vi "MecaDrivePoseEst_New.vi"(4 "WheelPositions":T1 {"RearRight" format="%19.3f"; "RearLeft" format="%19.3f"; "FrontRight" format="%19.3f"; "FrontLeft" format="%19.3f"}, 5 "gyroAngle":T6={"VALUE"=0.0, "COS"=1.0, "SIN"=0.0} {"SIN" format="%13.4f"; "COS" format="%13.4f"; "VALUE" format="%13.4f"}, 6 "MecanumKinematics":T2={"FrontLeft"={"X"=0.0, "Y"=0.0}, "FrontRight"={"X"=0.0, "Y"=0.0}, "RearLeft"={"X"=0.0, "Y"=0.0}, "RearRight"={"X"=0.0, "Y"=0.0}, "InverseKinematics"=[[0.0, 1.0, -1.0, 0.0], [0.0, 1.0, 1.0, 0.0], [0.0, 1.0, 1.0, 0.0], [0.0, 1.0, -1.0, 0.0]], "ForwardKinematics"=[[0.0, 1.0, -1.0, 0.0], [0.0, 1.0, 1.0, 0.0], [0.0, 1.0, 1.0, 0.0], [0.0, 1.0, -1.0, 0.0]], "PrevCoR"={"X"=0.0, "Y"=0.0}} {"PrevCoR"."Y" format="%14.3f"; "PrevCoR"."X" format="%14.3f"; "RearRight"."Y" format="%14.3f"; "RearRight"."X" format="%14.3f"; "RearLeft"."Y" format="%14.3f"; "RearLeft"."X" format="%14.3f"; "FrontRight"."Y" format="%14.3f"; "FrontRight"."X" format="%14.3f"; "FrontLeft"."Y" format="%14.3f"; "FrontLeft"."X" format="%14.3f"}, 7 "InitialPose":T5={"TRANSLATION"={"X"=0.0, "Y"=0.0}, "ROTATION"={"VALUE"=0.0, "COS"=1.0, "SIN"=0.0}} {"ROTATION"."SIN" format="%13.4f"; "ROTATION"."COS" format="%13.4f"; "ROTATION"."VALUE" format="%13.4f"; "TRANSLATION"."Y" format="%14.3f"; "TRANSLATION"."X" format="%14.3f"}, 8 "dt_Seconds":dbl=0.02, 9 "VisionMeasurementStdDevs":T4=[[0.0], [0.0], [0.0]], 10 "LocalMeasurementStdDevs":T4=[[0.0], [0.0], [0.0], [0.0], [0.0]], 11 "StateStdDevs":T4=[[0.0], [0.0], [0.0], [0.0], [0.0], [0.0], [0.0]]) -> (0 "Error":errorcluster, 3 "MecaDrivePoseEstimate":T7={"M_VisionContR"=[], "m_nominal_dT"=0.0, "m_PrevTime_Sec"=0.0, "m_GyroOffset"={"VALUE"=0.0, "COS"=1.0, "SIN"=0.0}, "m_PrevAngle"={"VALUE"=0.0, "COS"=1.0, "SIN"=0.0}, "m_Observer"={"m_P"=[], "m_xHat"=[], "States"=0, "Outputs"=0, "m_ContR"=[], "m_ContQ"=[], "m_SigmasF"=[], "m_dT_Sec"=0.0, "MERWE_SCALED_SIGMA_PTS"={"m_Wm"=[], "States"=0, "Alpha"=0.0, "m_Wc"=[], "Kappa"=0}, "meanFuncX"=refnum, "meanFuncY"=refnum, "residualFuncX"=refnum, "residualFuncY"=refnum, "addFuncX"=refnum, "addFuncXExtra"=variant, "residualFuncYExtra"=variant, "residualFuncXExtra"=variant, "MeanFuncYExtra"=variant, "MeanFuncXExtra"=variant, "Inputs"=0}, "m_kinematics"={"FrontLeft"={"X"=0.0, "Y"=0.0}, "FrontRight"={"X"=0.0, "Y"=0.0}, "RearLeft"={"X"=0.0, "Y"=0.0}, "RearRight"={"X"=0.0, "Y"=0.0}, "InverseKinematics"=[[0.0, 1.0, -1.0, 0.0], [0.0, 1.0, 1.0, 0.0], [0.0, 1.0, 1.0, 0.0], [0.0, 1.0, -1.0, 0.0]], "ForwardKinematics"=[[0.0, 1.0, -1.0, 0.0], [0.0, 1.0, 1.0, 0.0], [0.0, 1.0, 1.0, 0.0], [0.0, 1.0, -1.0, 0.0]], "PrevCoR"={"X"=0.0, "Y"=0.0}}, "Pose_Buffer"={"TimeStamps"=[], "Pose"=[], "Min_TimeStamp"=0.0, "Max_TimeStamp"=0.0, "ItemCount"=0, "MaxBufferTime"=0.0}} {"Pose_Buffer"."Pose"."ROTATION"."SIN" format="%13.4f"; "Pose_Buffer"."Pose"."ROTATION"."COS" format="%13.4f"; "Pose_Buffer"."Pose"."ROTATION"."VALUE" format="%13.4f"; "Pose_Buffer"."Pose"."TRANSLATION"."Y" format="%14.3f"; "Pose_Buffer"."Pose"."TRANSLATION"."X" format="%14.3f"; "m_kinematics"."PrevCoR"."Y" format="%14.3f"; "m_kinematics"."PrevCoR"."X" format="%14.3f"; "m_kinematics"."RearRight"."Y" format="%14.3f"; "m_kinematics"."RearRight"."X" format="%14.3f"; "m_kinematics"."RearLeft"."Y" format="%14.3f"; "m_kinematics"."RearLeft"."X" format="%14.3f"; "m_kinematics"."FrontRight"."Y" format="%14.3f"; "m_kinematics"."FrontRight"."X" format="%14.3f"; "m_kinematics"."FrontLeft"."Y" format="%14.3f"; "m_kinematics"."FrontLeft"."X" format="%14.3f"; "m_PrevAngle"."SIN" format="%13.4f"; "m_PrevAngle"."COS" format="%13.4f"; "m_PrevAngle"."VALUE" format="%13.4f"; "m_GyroOffset"."SIN" format="%13.4f"; "m_GyroOffset"."COS" format="%13.4f"; "m_GyroOffset"."VALUE" format="%13.4f"})   [LabVIEW 2019, in "Trajectory_Library.lvlib"]
doc: "Constructs a MecaDrivePoseEstimator.\n\nThis data cluster and its associated function blocks wrap an UnscentedKalmanFilter Unscented Kalman Filter to fuse latency-compensated vision measurements with mecanum drive encoder velocity measurements. It will correct for noisy measurements and encoder drift. It is intended to be an easy but more accurate drop-in for MecanumDriveOdometry.\n \nMecanumDrivePoseEstimator_update should be called every robot loop. If your loops are faster or slower than the default of 20 ms, then you should change the nominal delta time using the secondary constructor: MecanumDrivePoseEstimator_MecanumDrivePoseEstimator(Rotation2d, Pose2d MecanumDriveWheelPositions, MecanumDriveKinematics, Matrix, Matrix, Matrix, double).\n \nMecanumDrivePoseEstimator_addVisionMeasurement can be called as infrequently as you want; if you never call it, then this data cluster will behave mostly like regular encoder odometry.\n \nThe state-space system used internally has the following states (x), inputs (u), and outputs (y):\n \n x = [x, y, theta, s_fl, s_fr, s_rl, s_rr]T \n\n in the field coordinate system containing x position, y position, and heading, followed by\n the distance driven by the front left, front right, rear left, and rear right wheels.\n \n u = [v_x, v_y, omega, v_fl, v_fr, v_rl, v_rr]T \n\n containing x velocity, y velocity, and angular rate in the field coordinate system, \n followed by the velocity of the front left, front right, rear left, and rear right wheels.\n \n y = [x, y, theta]T \n\n from vision containing x position, y position, and heading; or \n\n y = [theta, s_fl, s_fr, s_rl, s_rr]T\n\n containing gyro heading, followed by the distance driven by the front left, front \n right, rear left, and rear right wheels.\n \nInputs: \n - gyroAngle -- The current gyro angle.\n - initialPoseMeters -- The starting pose estimate.\n - wheelPositions -- The distances driven by each wheel.\n - kinematics -- A correctly-configured kinematics object for your drivetrain.\n - stateStdDevs -- Standard deviations of model states. Increase these numbers\n to trust your model's state estimates less. This matrix is in the\n form [x, y, theta, s_fl, s_fr, s_rl, s_rr]T, with units in meters \n and radians, followed by meters.\n - localMeasurementStdDevs -- Standard deviation of the gyro measurement. \n Increase this number to trust sensor readings from the gyro less. \n This matrix is in the form [theta, s_fl, s_fr, s_rl, s_rr], with \n units in radians, followed by meters.\n - visionMeasurementStdDevs -- Standard deviations of the vision measurements. \n Increase these numbers to trust global measurements from vision \n less. This matrix is in the form [x, y, theta]T, with units in \n meters and radians.\n - nominalDtSeconds -- The time in seconds between each robot loop.\n\nOutputs:\n - outMecaPoseEst -- Updated data cluster \n - Error -- If TRUE, an error occured."
uses:
  Trajectory_Library.lvlib
  <vilib>/Analysis/Matrix/Datatypes/RealMatrix.ctl
  <vilib>/Analysis/Matrix/NI_Matrix.lvlib
  TypeDef/MERWE_SCALED_SIGMA_PTS.ctl
  TypeDef/UNSCENTED_KALMAN_FILTER.ctl
  TypeDef/CALLBACK_FUNC_TYPE.ctl
  TypeDef/ROTATION2D.ctl
  TypeDef/TRANSLATION2D.ctl
  TypeDef/POSE2D.ctl
  TypeDef/TIME_INTERPOLATABLE_POSE2D.ctl
  TypeDef/MECA_DRIVE_KINEMATICS.ctl
  TypeDef/MECA_DRIVE_POSE_EST.ctl
  TypeDef/MECA_WHEEL_POSITIONS.ctl
panel:
  # "<7,1>"
  # "<5, 1>"
  # "<3, 1>"
  # "<3, 3>"
  # "State Estimate <Statess,1>"
  # "<States, States>"
  # "<States, ?>"
  # "<Statess,  States>"
  # "<Outputs, Outputs>"
  # "<?, 1>"
  # "<?, 1>"
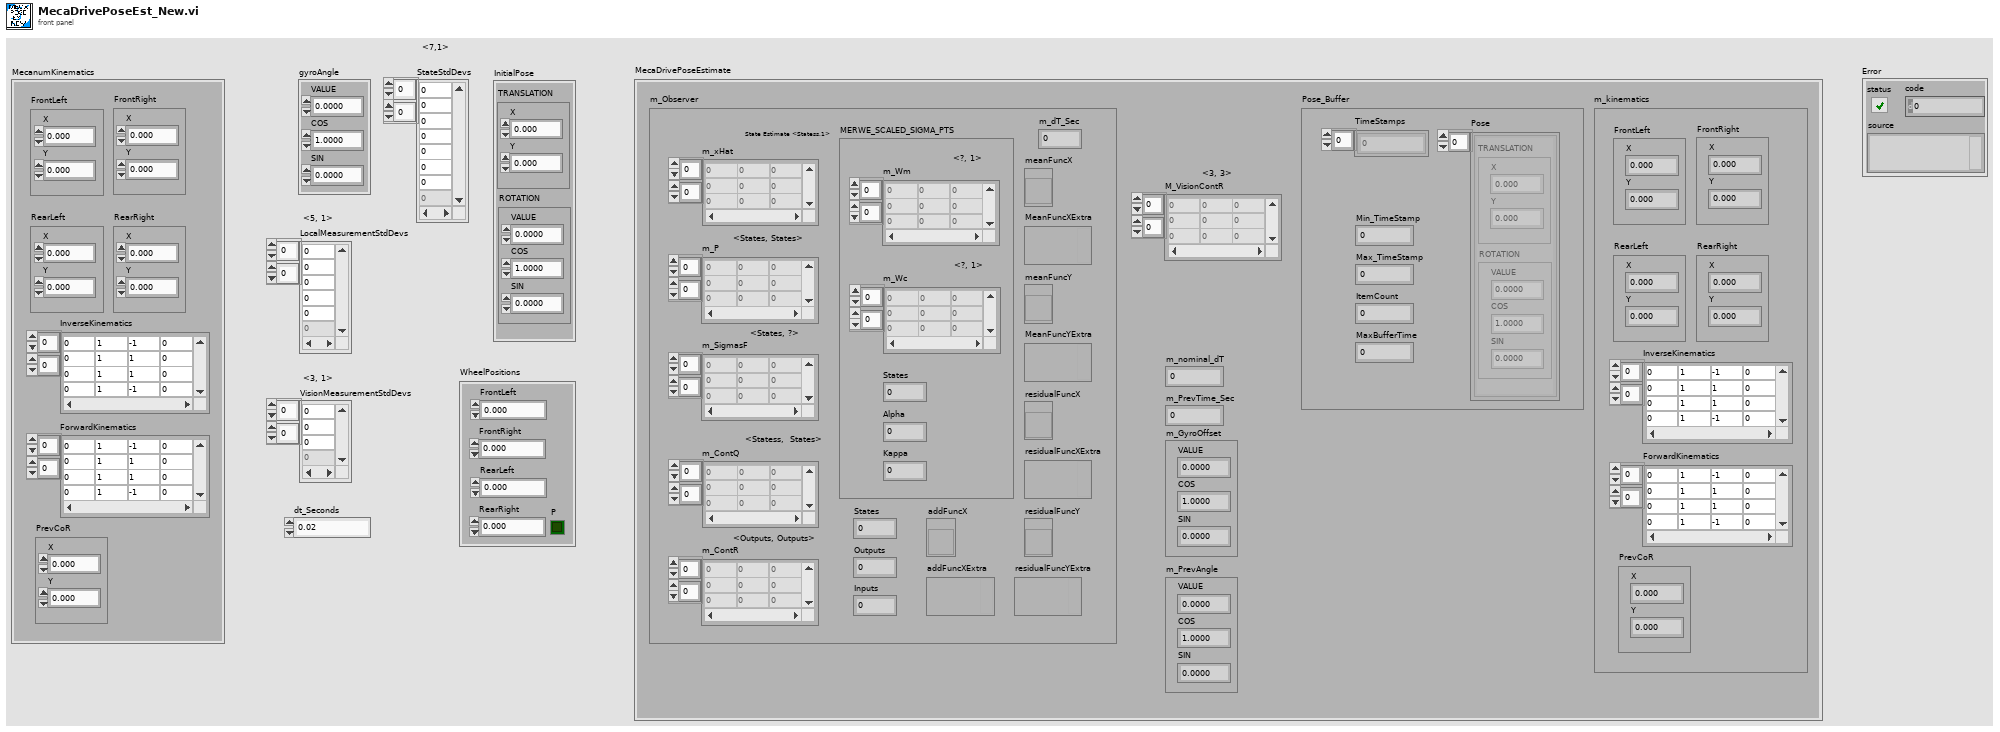
[diagram p1: front panel]
types:
  T1 = typedef "Trajectory_Library.lvlib/MECA_WHEEL_POSITIONS.ctl" = cluster{"FrontLeft":dbl, "FrontRight":dbl, "RearLeft":dbl, "RearRight":dbl, "P":bool}
  T2 = typedef "Trajectory_Library.lvlib/MECA_DRIVE_KINEMATICS.ctl" = cluster{"FrontLeft":T3, "FrontRight":T3, "RearLeft":T3, "RearRight":T3, "InverseKinematics":T4, "ForwardKinematics":T4, "PrevCoR":T3}
  T3 = typedef "Trajectory_Library.lvlib/TRANSLATION2D.ctl" = cluster{"X":dbl, "Y":dbl}
  T4 = typedef "NI_Matrix.lvlib/RealMatrix.ctl" = dbl[][]
  T5 = typedef "Trajectory_Library.lvlib/POSE2D.ctl" = cluster{"TRANSLATION":T3, "ROTATION":T6}
  T6 = typedef "Trajectory_Library.lvlib/ROTATION2D.ctl" = cluster{"VALUE":dbl, "COS":dbl, "SIN":dbl}
  T7 = typedef "Trajectory_Library.lvlib/MECA_DRIVE_POSE_EST.ctl" = cluster{"M_VisionContR":T4, "m_nominal_dT":dbl, "m_PrevTime_Sec":dbl, "m_GyroOffset":T6, "m_PrevAngle":T6, "m_Observer":T8, "m_kinematics":T2, "Pose_Buffer":T11}
  T8 = typedef "Trajectory_Library.lvlib/UNSCENTED_KALMAN_FILTER.ctl" = cluster{"m_P":T4, "m_xHat":T4, "States":i32, "Outputs":i32, "m_ContR":T4, "m_ContQ":T4, "m_SigmasF":T4, "m_dT_Sec":dbl, "MERWE_SCALED_SIGMA_PTS":T9, "meanFuncX":T10, "meanFuncY":T10, "residualFuncX":T10, "residualFuncY":T10, "addFuncX":T10, "addFuncXExtra":variant, "residualFuncYExtra":variant, "residualFuncXExtra":variant, "MeanFuncYExtra":variant, "MeanFuncXExtra":variant, "Inputs":i32}
  T9 = typedef "Trajectory_Library.lvlib/MERWE_SCALED_SIGMA_PTS.ctl" = cluster{"m_Wm":T4, "States":i32, "Alpha":dbl, "m_Wc":T4, "Kappa":i32}
  T10 = typedef "Trajectory_Library.lvlib/CALLBACK_FUNC_TYPE.ctl" = refnum<vi>
  T11 = typedef "Trajectory_Library.lvlib/TIME_INTERPOLATABLE_POSE2D.ctl" = cluster{"TimeStamps":dbl[], "Pose":T5[], "Min_TimeStamp":dbl, "Max_TimeStamp":dbl, "ItemCount":i32, "MaxBufferTime":dbl}
  T12 = typedef "Trajectory_Library.lvlib/UNSCENTED_KALMAN_NEW_FUNC_GROUP.ctl" = cluster{"meanFuncX":T10, "meanFuncY":T10, "residualFuncX":T10, "residualFuncY":T10, "addFuncX":T10, "MeanFuncXExtra":variant, "MeanFuncYExtra":variant, "residualFuncXExtra":variant, "residualFuncYExtra":variant, "addFuncXExtra":variant}
  T13 = typedef "WPILib_Math.lvlib/TIME_INTERPOLATABLE_POSE2D.ctl" = cluster{"TimeStamps":dbl[], "Pose":T14[], "Min_TimeStamp":dbl, "Max_TimeStamp":dbl, "ItemCount":i32, "MaxBufferTime":dbl}
  T14 = typedef "WPILib_Math.lvlib/POSE2D.ctl" = cluster{"TRANSLATION":T15, "ROTATION":T16}
  T15 = typedef "WPILib_Math.lvlib/TRANSLATION2D.ctl" = cluster{"X":dbl, "Y":dbl}
  T16 = typedef "WPILib_Math.lvlib/ROTATION2D.ctl" = cluster{"VALUE":dbl, "COS":dbl, "SIN":dbl}
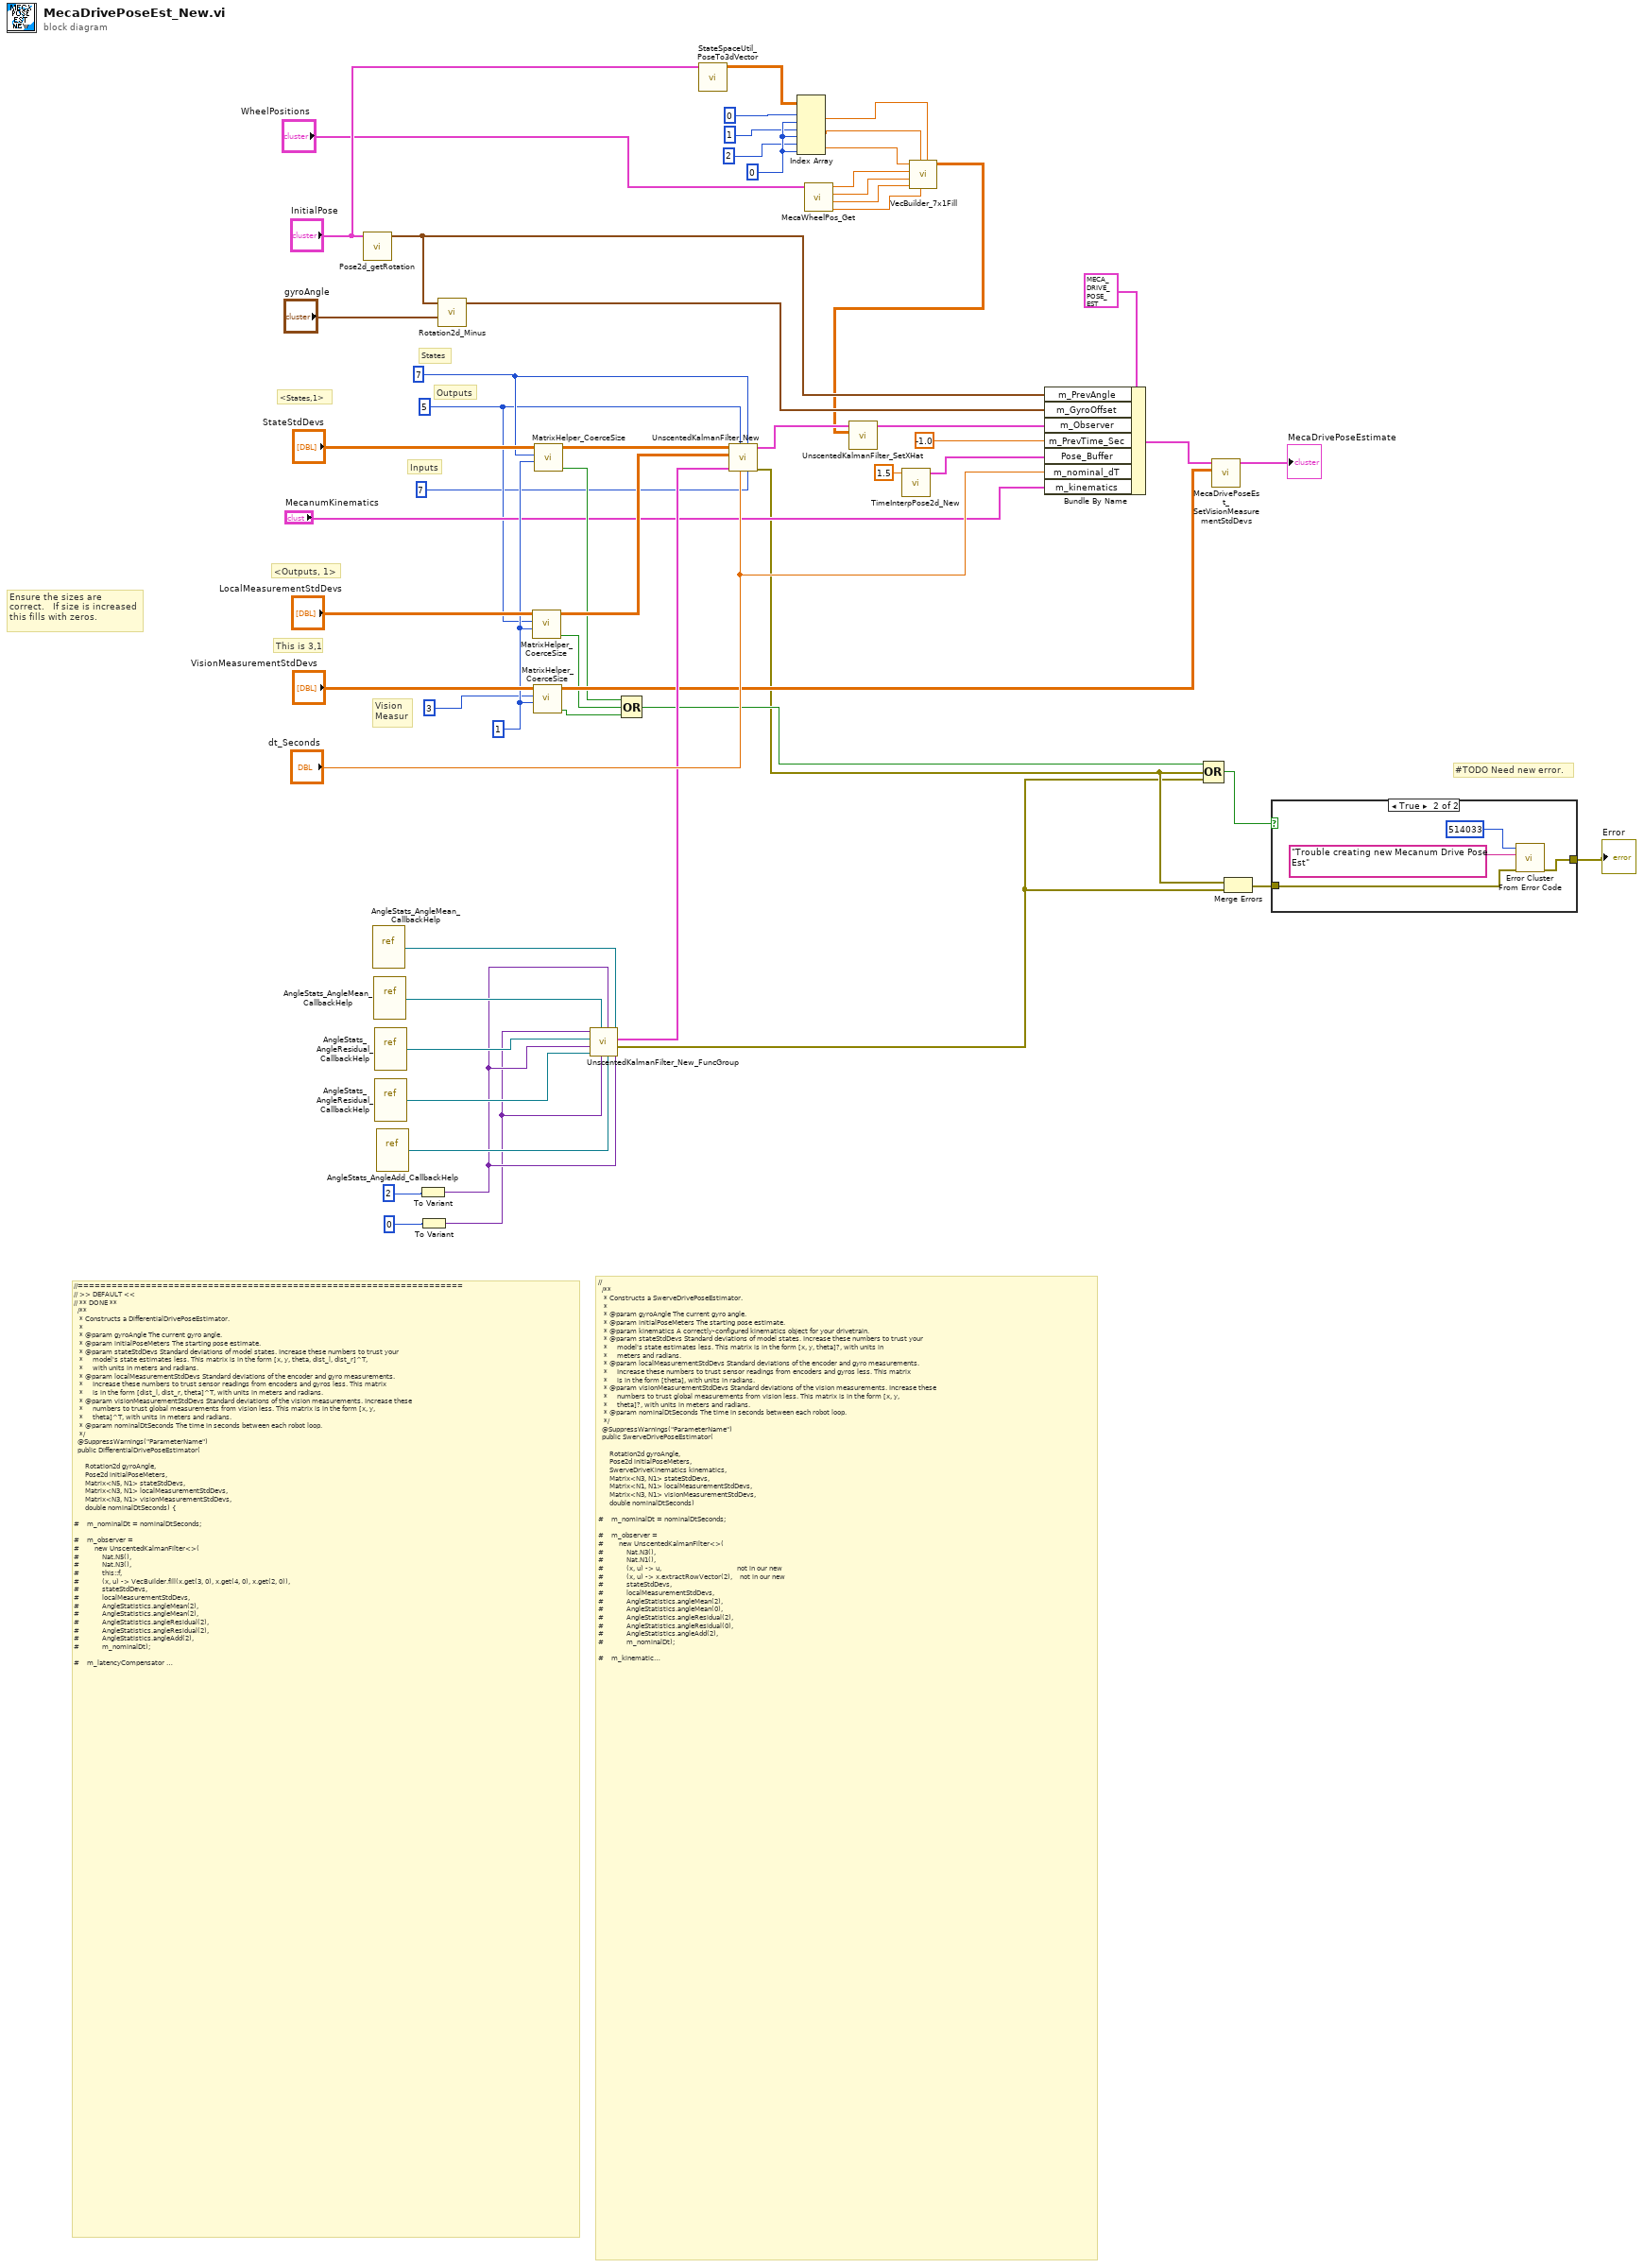
[diagram p0: block diagram]
diagram:
  w12 = 0 ("index (col)")
  w34 = 1 ("y")
  w25 = 5 ("Outputs")
  w33 = 7 ("States")
  # "Vision\nMeasur"
  # "#TODO Need new error."
  # "This is 3,1"
  # "//====================================================================\n// >> DEFAULT <<\n// ** DONE **\n  /**\n   * Constructs a DifferentialDrivePoseEstimator.\n   *\n   * @param gyroAngle The current gyro angle.\n   * @param initialPoseMeters The starting pose estimate.\n   * @param stateStdDevs Standard deviations of model states. Increase these numbers to trust your\n   *     model's state estimates less. This matrix is in the form [x, y, theta, dist_l, dist_r]^T,\n   *     with units in meters and radians.\n   * @param localMeasurementStdDevs Standard deviations of the encoder and gyro measurements.\n   *     Increase these numbers to trust sensor readings from encoders and gyros less. This matrix\n   *     is in the form [dist_l, dist_r, theta]^T, with units in meters and radians.\n   * @param visionMeasurementStdDevs Standard deviations of the vision measurements. Increase these\n   *     numbers to trust global measurements from vision less. This matrix is in the form [x, y,\n   *     theta]^T, with units in meters and radians.\n   * @param nominalDtSeconds The time in seconds between each robot loop.\n   */\n  @SuppressWarnings(\"ParameterName\")\n  public DifferentialDrivePoseEstimator(\n\n      Rotation2d gyroAngle,\n      Pose2d initialPoseMeters,\n      Matrix<N5, N1> stateStdDevs,\n      Matrix<N3, N1> localMeasurementStdDevs,\n      Matrix<N3, N1> visionMeasurementStdDevs,\n      double nominalDtSeconds) {\n\n#    m_nominalDt = nominalDtSeconds;\n\n#    m_observer =\n#        new UnscentedKalmanFilter<>(\n#            Nat.N5(),\n#            Nat.N3(),\n#            this::f,\n#            (x, u) -> VecBuilder.fill(x.get(3, 0), x.get(4, 0), x.get(2, 0)),\n#            stateStdDevs,\n#            localMeasurementStdDevs,\n#            AngleStatistics.angleMean(2),\n#            AngleStatistics.angleMean(2),\n#            AngleStatistics.angleResidual(2),\n#            AngleStatistics.angleResidual(2),\n#            AngleStatistics.angleAdd(2),\n#            m_nominalDt);\n\n#    m_latencyCompensator = new KalmanFilterLatencyCompensator<>();\n\n#    // Initialize vision R\n#    setVisionMeasurementStdDevs(visionMeasurementStdDevs);\n\n//JAS not part of the data structure....\n    m_visionCorrect =\n        (u, y) ->\n            m_observer.correct(\n                Nat.N3(),\n                u,\n                y,\n                (x, u1) -> new Matrix<>(x.getStorage().extractMatrix(0, 3, 0, 1)),\n                m_visionDiscreteR,\n                AngleStatistics.angleMean(2),\n                AngleStatistics.angleResidual(2),\n                AngleStatistics.angleResidual(2),\n                AngleStatistics.angleAdd(2));\n\n#    m_gyroOffset = initialPoseMeters.getRotation().minus(gyroAngle);\n#    m_previousAngle = initialPoseMeters.getRotation();\n#    m_observer.setXhat(fillStateVector(initialPoseMeters, 0.0, 0.0));\n  }"
  # "// \n  /**\n   * Constructs a SwerveDrivePoseEstimator.\n   *\n   * @param gyroAngle The current gyro angle.\n   * @param initialPoseMeters The starting pose estimate.\n   * @param kinematics A correctly-configured kinematics object for your drivetrain.\n   * @param stateStdDevs Standard deviations of model states. Increase these numbers to trust your\n   *     model's state estimates less. This matrix is in the form [x, y, theta]?, with units in\n   *     meters and radians.\n   * @param localMeasurementStdDevs Standard deviations of the encoder and gyro measurements.\n   *     Increase these numbers to trust sensor readings from encoders and gyros less. This matrix\n   *     is in the form [theta], with units in radians.\n   * @param visionMeasurementStdDevs Standard deviations of the vision measurements. Increase these\n   *     numbers to trust global measurements from vision less. This matrix is in the form [x, y,\n   *     theta]?, with units in meters and radians.\n   * @param nominalDtSeconds The time in seconds between each robot loop.\n   */\n  @SuppressWarnings(\"ParameterName\")\n  public SwerveDrivePoseEstimator(\n\n      Rotation2d gyroAngle,\n      Pose2d initialPoseMeters,\n      SwerveDriveKinematics kinematics,\n      Matrix<N3, N1> stateStdDevs,\n      Matrix<N1, N1> localMeasurementStdDevs,\n      Matrix<N3, N1> visionMeasurementStdDevs,\n      double nominalDtSeconds) \n\n#    m_nominalDt = nominalDtSeconds;\n\n#    m_observer =\n#        new UnscentedKalmanFilter<>(\n#            Nat.N3(),\n#            Nat.N1(),\n#            (x, u) -> u,                                        not in our new\n#            (x, u) -> x.extractRowVector(2),    not in our new\n#            stateStdDevs,\n#            localMeasurementStdDevs,\n#            AngleStatistics.angleMean(2),\n#            AngleStatistics.angleMean(0),\n#            AngleStatistics.angleResidual(2),\n#            AngleStatistics.angleResidual(0),\n#            AngleStatistics.angleAdd(2),\n#            m_nominalDt);\n\n#    m_kinematics = kinematics;\n\n#    m_latencyCompensator = new KalmanFilterLatencyCompensator<>();\n\n#    // Initialize vision R\n#    setVisionMeasurementStdDevs(visionMeasurementStdDevs);\n\n//JAS not part of the data structure....\n    m_visionCorrect =\n        (u, y) ->\n            m_observer.correct(\n                Nat.N3(),\n                u,\n                y,\n                (x, u1) -> x,\n                m_visionContR,\n                AngleStatistics.angleMean(2),\n                AngleStatistics.angleResidual(2),\n                AngleStatistics.angleResidual(2),\n                AngleStatistics.angleAdd(2));\n\n#    m_gyroOffset = initialPoseMeters.getRotation().minus(gyroAngle);\n#    m_previousAngle = initialPoseMeters.getRotation();\n#    m_observer.setXhat(  StateSpaceUtil.poseTo3dVector(initialPoseMeters));\n  }"
  # "Inputs"
  # "Outputs"
  # "States"
  # "<Outputs, 1>"
  # "<States,1>"
  # "Ensure the sizes are\ncorrect.   If size is increased \nthis fills with zeros."
  n1 = call "Pose2d_getRotation.vi"("in POSE"="InitialPose") -> ("out ROTATION"=w54:T6)  [unwired: 10 in]
  n2 = vi-ref "AngleStats_AngleMean_CallbackHelp.vi"() -> (w47:refnum<vi>)
  n3 = vi-ref "AngleStats_AngleMean_CallbackHelp.vi"() -> (w46:refnum<vi>)
  n4 = vi-ref "AngleStats_AngleResidual_CallbackHelp.vi"() -> (w45:refnum<vi>)
  n5 = vi-ref "AngleStats_AngleResidual_CallbackHelp.vi"() -> (w44:refnum<vi>)
  n6 = vi-ref "AngleStats_AngleAdd_CallbackHelp.vi"() -> (w42:refnum<vi>)
  n7 = To Variant(anything=2) -> (Variant=w41:variant)
  n8 = To Variant(anything=0) -> (Variant=w27:variant)
  n9 = call "Rotation2d_Minus.vi"("other ROTATION"="gyroAngle", "in ROTATION"=w54) -> ("out ROTATION"=w55:T6)  [unwired: 9 in]
  n10 = call "MatrixHelper_CoerceSize.vi"("Columns"=w34, "Rows"=w25, "input matrix"="LocalMeasurementStdDevs") -> ("Coerced"=w30:bool, "output matrix"=w39:T4)  [unwired: 7 in]
  n11 = call "MatrixHelper_CoerceSize.vi"("Columns"=w34, "Rows"=3 ("Inputs"), "input matrix"="VisionMeasurementStdDevs") -> ("Coerced"=w29:bool, "output matrix"=w35:T4)  [unwired: 7 in]
  n12 = call "MatrixHelper_CoerceSize.vi"("Columns"=w34, "Rows"=w33, "input matrix"="StateStdDevs") -> ("Coerced"=w31:bool, "output matrix"=w37:T4)  [unwired: 7 in]
  n13 = call "UnscentedKalmanFilter_New_FuncGroup.vi"("addFuncXExtra"=w41, "MeanFuncX"=w47, "AddFuncX"=w42, "MeanFuncXExtra"=w41, "residualFuncYExtra"=w27, "MeanFuncY"=w46, "ResidualFuncY"=w44, "residualFuncXExtra"=w41, "ResidualFuncX"=w45, "MeanFuncYExtra"=w27) -> ("Error"=w19:errorcluster, "UNSCENTED_KALMAN_NEW_FUNC_GROUP"=w48:T12)
  n14 = Compound Arithmetic op=OR(w31, w30, w29) -> (w32:bool)
  n15 = call "StateSpaceUtil_PoseTo3dVector.vi"("Pose"="InitialPose") -> ("Pose Vector"=w14:T4)  [unwired: 10 in]
  n16 = call "UnscentedKalmanFilter_New.vi"("Inputs"=7, "States"=w33, "dt_Seconds"="dt_Seconds", "Outputs"=w25, "UNSCENTED_KALMAN_NEW_FUNC_GROUP"=w48, "MeasurementStdDevs"=w39, "StateStdDevs"=w37) -> ("Error"=w20:errorcluster, "UnscentedKalmanFiilter"=w52:T8)  [unwired: 3 in]
  n17 = Index Array(array=w14, index (row) #1=0 ("index (row)"), index (col) #1=w12, index (row) #2=1 ("index (row)"), index (col) #2=w12, index (row) #3=2 ("index (row)"), index (col) #3=w12) -> (element #1=w9:dbl, element #2=w8:dbl, element #3=w7:dbl)
  n18 = call "MecaWheelPos_Get.vi"("MECA_WHEEL_POSITIONS"="WheelPositions") -> ("RearRightPosition"=w3:dbl, "RearLeftPosition"=w4:dbl, "FrontRightPosition"=w5:dbl, "FrontLeftPosition"=w6:dbl)  [unwired: 7 in]
  n19 = call "TimeInterpPose2d_New.vi"("MaxTime"=1.5) -> ("TimeInterpPose"=w16:T13)  [unwired: 10 in]
  n20 = call "VecBuilder_7x1Fill.vi"("R0"=w9, "R6"=w3, "R1"=w8, "R5"=w4, "R4"=w5, "R3"=w6, "R2"=w7) -> ("output matrix"=w1:T4)  [unwired: 4 in]
  n21 = call "UnscentedKalmanFilter_SetXHat.vi"("xHat"=w1, "in UnscentedKalmanFiilter"=w52) -> ("out UnscentedKalmanFiilter"=w53:T8)  [unwired: 8 in, 1 out]
  n22 = Bundle By Name(cluster=T7 {"M_VisionContR"=[], "m_nominal_dT"=0.0, "m_PrevTime_Sec"=0.0, "m_GyroOffset"={"VALUE"=0.0, "COS"=1.0, "SIN"=0.0}, "m_PrevAngle"={"VALUE"=0.0, "COS"=1.0, "SIN"=0.0}, "m_Observer"={"m_P"=[], "m_xHat"=[], "States"=0, "Outputs"=0, "m_ContR"=[], "m_ContQ"=[], "m_SigmasF"=[], "m_dT_Sec"=0.0, "MERWE_SCALED_SIGMA_PTS"={"m_Wm"=[], "States"=0, "Alpha"=0.0, "m_Wc"=[], "Kappa"=0}, "meanFuncX"=refnum, "meanFuncY"=refnum, "residualFuncX"=refnum, "residualFuncY"=refnum, "addFuncX"=refnum, "addFuncXExtra"=variant, "residualFuncYExtra"=variant, "residualFuncXExtra"=variant, "MeanFuncYExtra"=variant, "MeanFuncXExtra"=variant, "Inputs"=0}, "m_kinematics"={"FrontLeft"={"X"=0.0, "Y"=0.0}, "FrontRight"={"X"=0.0, "Y"=0.0}, "RearLeft"={"X"=0.0, "Y"=0.0}, "RearRight"={"X"=0.0, "Y"=0.0}, "InverseKinematics"=[[0.0, 1.0, -1.0, 0.0], [0.0, 1.0, 1.0, 0.0], [0.0, 1.0, 1.0, 0.0], [0.0, 1.0, -1.0, 0.0]], "ForwardKinematics"=[[0.0, 1.0, -1.0, 0.0], [0.0, 1.0, 1.0, 0.0], [0.0, 1.0, 1.0, 0.0], [0.0, 1.0, -1.0, 0.0]], "PrevCoR"={"X"=0.0, "Y"=0.0}}, "Pose_Buffer"={"TimeStamps"=[], "Pose"=[], "Min_TimeStamp"=0.0, "Max_TimeStamp"=0.0, "ItemCount"=0, "MaxBufferTime"=0.0}} ("DIFF_DRIVE_POSE_EST"), "m_PrevAngle"=w54, "m_GyroOffset"=w55, "m_Observer"=w53, "m_PrevTime_Sec"=-1.0, "Pose_Buffer"=w16, "m_nominal_dT"="dt_Seconds", "m_kinematics"="MecanumKinematics") -> (w51:T7)
  n23 = Compound Arithmetic op=OR(w32, w20, w19) -> (w21:bool)
  n24 = call "MecaDrivePoseEst_SetVisionMeasurementStdDevs.vi"("VisionMeasurementStdDevs"=w35, "in MecaDrivePoseEstimate"=w51) -> ("Out MecaDrivePoseEstimate"=→"MecaDrivePoseEstimate":T7)  [unwired: 8 in, 1 out]
  n25 = Merge Errors(w20, w19) -> (w22:errorcluster)
  n26 = case shown="True" w21 {
    tunnel: w22 -> [w59 w62]
    tunnel: [w59 w63] -> w18
    frame False {
    }
    frame True {
      n27 = call <vilib>:"Error Cluster From Error Code.vi"("error in (no error)"=w62, "error message (\"\")"="Trouble creating new Mecanum Drive Pose Est" ("error message (\"\")"), "error code (0)"=514033) -> ("error out"=w63:errorcluster)  [unwired: 6 in]
    }
  }
  "Error" <- w18
